vi "testRun.vi"() -> ()   [LabVIEW 2025, in "FRtest.lvclass"]
uses:
  FRtest.lvclass
  H1 Frequency Response.lvclass
  <vilib>/measure/NI_MABase.lvlib
panel:
  in  "loop":u32=50
  # "Not exceed 50 ms"
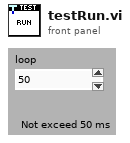
[diagram p1: front panel]
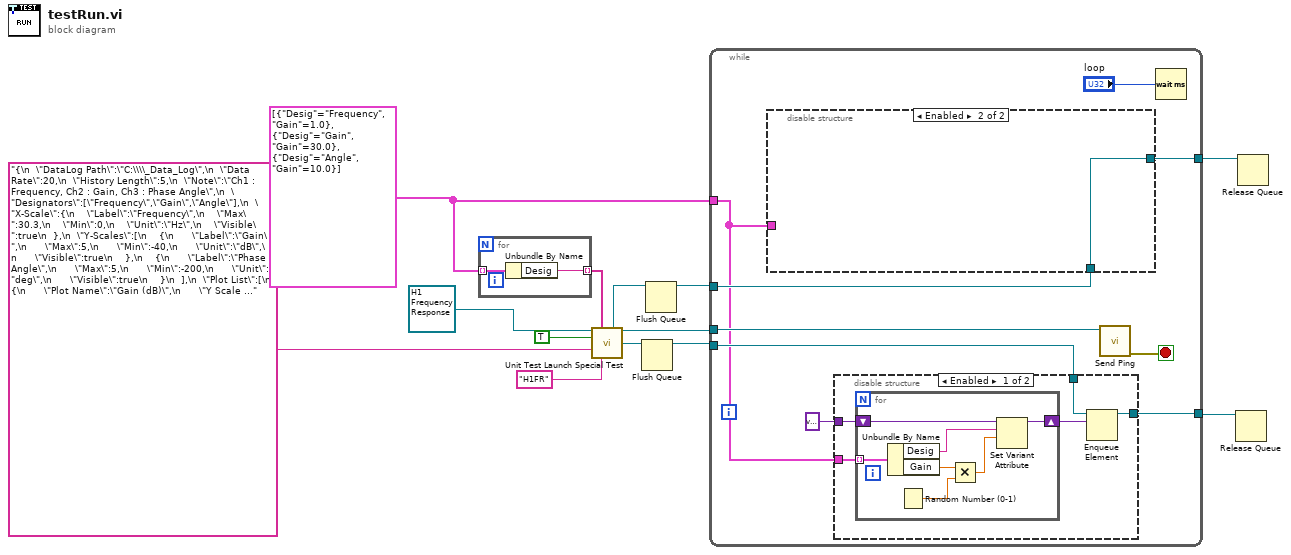
[diagram p0: block diagram]
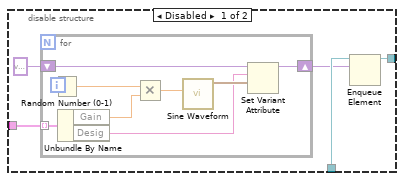
[diagram p2: hidden frame]
diagram:
  w1 = cluster{"Desig":string, "Gain":dbl}[] [{"Desig"="Frequency", "Gain"=1.0}, {"Desig"="Gain", "Gain"=30.0}, {"Desig"="Angle", "Gain"=10.0}] ("Sim Param")
  n1 = for {
    tunnel: w1 -> [w15] mode=indexing
    tunnel: [w14] -> w10 mode=indexing
    n2 = Unbundle By Name(w15) -> ("Desig"=w14:string)
  }
  n3 = call "Unit Test Launch Special Test.vi"("Special Test Class"=refnum<class "H1 Frequency Response.lvclass"> refnum ("Sensitivity.lvlib:Sensitivity.lvclass"), "Subscription Alias"=w10, "Auto Launched"=TRUE, "<JSON>"="{\n  \"DataLog Path\":\"C:\\\\_Data_Log\",\n  \"Data Rate\":20,\n  \"History Length\":5,\n  \"Note\":\"Ch1 : Frequency, Ch2 : Gain, Ch3 : Phase Angle\",\n  \"Designators\":[\"Frequency\",\"Gain\",\"Angle\"],\n  \"X-Scale\":{\n    \"Label\":\"Frequency\",\n    \"Max\":30.3,\n    \"Min\":0,\n    \"Unit\":\"Hz\",\n    \"Visible\":true\n  },\n  \"Y-Scales\":[\n    {\n      \"Label\":\"Gain\",\n      \"Max\":5,\n      \"Min\":-40,\n      \"Unit\":\"dB\",\n      \"Visible\":true\n    },\n    {\n      \"Label\":\"Phase Angle\",\n      \"Max\":5,\n      \"Min\":-200,\n      \"Unit\":\"deg\",\n      \"Visible\":true\n    }\n  ],\n  \"Plot List\":[\n    {\n      \"Plot Name\":\"Gain (dB)\",\n      \"Y Scale Index\":0,\n      \"Visible\":true\n    },\n    {\n      \"Plot Name\":\"Phase Angle (deg)\",\n      \"Y Scale Index\":1,\n      \"Visible\":true\n    }\n  ]\n}" ("Settings_JSON_"), "Debug Alias"="H1FR") -> ("Data Queue out"=w7:refnum<queue>, "ST Enqueuer out"=w2:refnum<class "Message Enqueuer.lvclass">, "Fast Map Queue out"=w8:refnum<queue>)  [unwired: 2 in, 6 out]
  n4 = Flush Queue(queue=w8) -> (queue out=w3:refnum<queue>)  [unwired: 1 in, 2 out]
  n5 = Flush Queue(queue=w7) -> (queue out=w4:refnum<queue>)  [unwired: 1 in, 2 out]
  n6 = while {
    tunnel: w2 -> [w24]
    tunnel: w3 -> [w21]
    tunnel: [w19] -> w5
    tunnel: w1 -> [w18]
    tunnel: w4 -> [w23]
    tunnel: [w20] -> w6
    stop <- w17 stop-if-true
    n7 = disable-structure shown="Enabled" {
      disable-tunnel: w23 -> [w28 w38]
      disable-tunnel: [w27 w38] -> w19
      disable-tunnel: w18 -> [w26 _]
      frame Disabled {
        n8 = for {
          shift-right: [w36] -> w25
          shift-left: variant ("variant") -> [w37]
          tunnel: w26 -> [w34] mode=indexing
          n9 = Random Number (0-1)() -> (number: 0 to 1=w30:dbl)
          n10 = Unbundle By Name(w34) -> ("Gain"=w32:dbl, "Desig"=w33:string)
          n11 = Multiply(x=w30, y=w32) -> (x*y=w31:dbl)
          n12 = call <vilib>:"Sine Waveform.vi"("amplitude"=w31) -> ("signal out"=w35:waveform(dbl))  [unwired: 9 in, 1 out]
          n13 = Set Variant Attribute(Variant=w37, name=w33, value=w35) -> (Variant out=w36:variant)  [unwired: 1 in, 2 out]
        }
        n14 = Enqueue Element(queue=w28, element=w25) -> (queue out=w27:refnum<queue>)  [unwired: 2 in, 2 out]
      }
      frame Enabled {
      }
    }
    n15 = disable-structure shown="Enabled" {
      disable-tunnel: variant ("variant") -> [w43 _]
      disable-tunnel: w21 -> [w42 w51]
      disable-tunnel: [w41 w51] -> w20
      disable-tunnel: w18 -> [w40 _]
      frame Enabled {
        n16 = for {
          shift-right: [w49] -> w39
          shift-left: w43 -> [w50]
          tunnel: w40 -> [w48] mode=indexing
          n17 = Unbundle By Name(w48) -> ("Desig"=w47:string, "Gain"=w46:dbl)
          n18 = Random Number (0-1)() -> (number: 0 to 1=w45:dbl)
          n19 = Multiply(x=w46, y=w45) -> (x*y=w44:dbl)
          n20 = Set Variant Attribute(Variant=w50, name=w47, value=w44) -> (Variant out=w49:variant)  [unwired: 1 in, 2 out]
        }
        n21 = Enqueue Element(queue=w42, element=w39) -> (queue out=w41:refnum<queue>)  [unwired: 2 in, 2 out]
      }
      frame Disabled {
      }
    }
    n22 = call "Send Ping.vi"("Message Enqueuer"=w24) -> ("error out"=w17:errorcluster)  [unwired: 6 in, 4 out]
    n23 = Wait (ms)(milliseconds to wait="loop") -> ()  [unwired: 1 out]
  }
  n24 = Release Queue(queue=w6) -> ()  [unwired: 2 in, 3 out]
  n25 = Release Queue(queue=w5) -> ()  [unwired: 2 in, 3 out]
